vi "Acquire Sine Block.vi"(8 "error in":errorcluster, 10 "start sample":dbl, 11 "generator settings":T1={"Amplitude"=1.0, "Frequency"=10.0, "Sample Rate"=1000.0, "Number of Samples"=1000, "Update Interval ms"=100}) -> (0 "error out":errorcluster, 2 "next start sample":dbl, 3 "waveform":cluster{"x_data":dbl[], "y_data":dbl[]})   [LabVIEW 2026, in "Sine Generator.lvlib"]
doc: "Acquisition stage. Produces the next block of the sine wave as an XY pair (time in seconds from 0, signal value) by calling the signal generation engine, and returns the sample index at which the next block starts: the start advances by sample rate x update interval, so consecutive updates scroll the signal at real-time speed."
uses:
  Sine Generator.lvlib
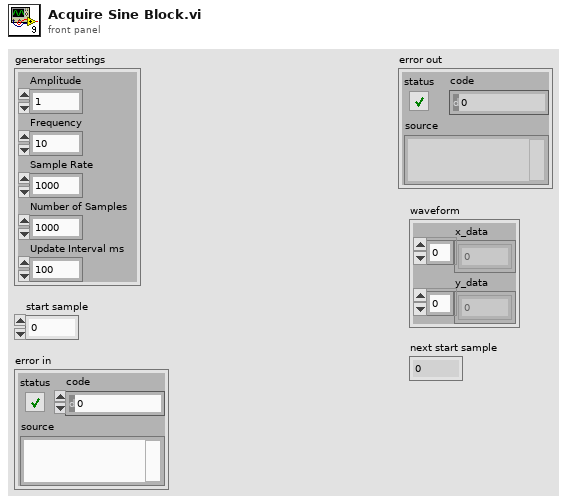
[diagram p1: front panel]
types:
  T1 = cluster{"Amplitude":dbl, "Frequency":dbl, "Sample Rate":dbl, "Number of Samples":i32, "Update Interval ms":i32}
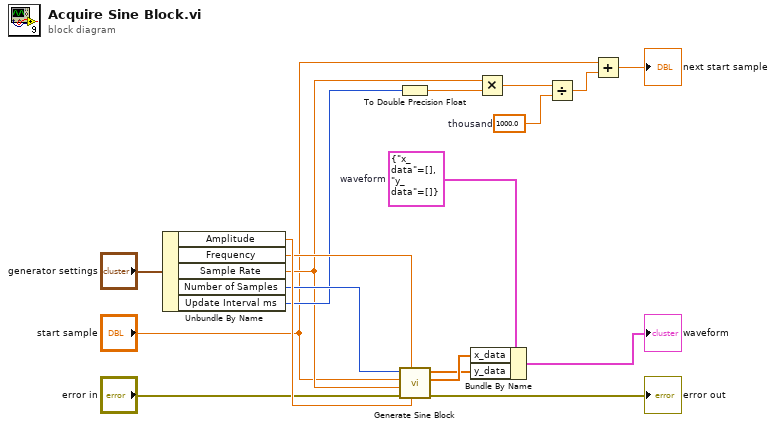
[diagram p0: block diagram]
diagram:
  w6 = 1000.0  # thousand
  w11 = cluster{"x_data":dbl[], "y_data":dbl[]} {"x_data"=[], "y_data"=[]}  # waveform
  n1 = Unbundle By Name("generator settings") -> ("Amplitude"=w17:dbl, "Frequency"=w16:dbl, "Sample Rate"=w9:dbl, "Number of Samples"=w14:i32, "Update Interval ms"=w10:i32)
  n2 = To Double Precision Float(number=w10) -> (double precision float=w8:dbl)
  n3 = call "Generate Sine Block.vi"("amplitude"=w17, "frequency"=w16, "error in"="error in", "sample rate"=w9, "start sample"="start sample", "samples"=w14) -> ("error out"=→"error out":errorcluster, "time"=w13:dbl[], "signal"=w12:dbl[])  [unwired: 3 in]
  n4 = Bundle By Name(cluster=w11, "x_data"=w13, "y_data"=w12) -> (→"waveform":cluster{"x_data":dbl[], "y_data":dbl[]})
  n5 = Multiply(x=w9, y=w8) -> (x*y=w7:dbl)
  n6 = Divide(x=w7, y=w6) -> (x/y=w4:dbl)
  n7 = Add(x="start sample", y=w4) -> (x+y=→"next start sample":dbl)
